vi "Set Description.vi"(8 "error in":errorcluster, 11 "ILabVIEWFile in":refnum<class "Type Definition.lvclass">) -> (0 "error out":errorcluster, 3 "ILabVIEWFile out":refnum<class "Type Definition.lvclass">)   [LabVIEW 2026, in "Type Definition.lvclass"]
doc: "Set description of labview file (vi or type definition)."
uses:
  Type Definition.lvclass
  Type Definition.lvclass/Type Definition.ctl
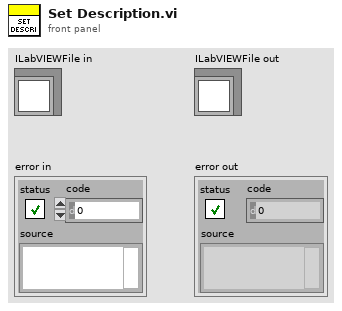
[diagram p1: front panel]
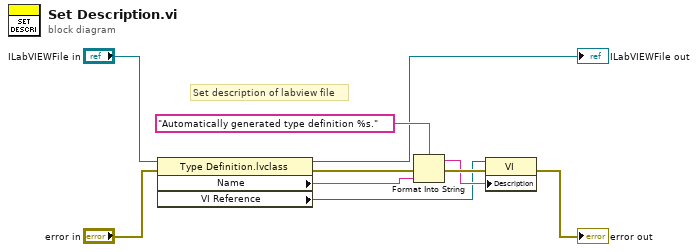
[diagram p0: block diagram]
diagram:
  # "Set description of labview file"
  n1 = property class="Type Definition.lvclass"(reference="ILabVIEWFile in", error in="error in") -> (reference out=→"ILabVIEWFile out":refnum<class "Type Definition.lvclass">, error out=w7:errorcluster, "Name"=w3:string, "VI Reference"=w1:refnum<vi>)
  n2 = Format Into String(format string="Automatically generated type definition %s.", error in=w7, w3) -> (resulting string=w5:string, error out=w9:errorcluster)  [unwired: 1 in]
  n3 = property on="Property Node" class="VI"(reference=w1, error in=w9, "Description"=w5) -> (error out=→"error out":errorcluster)  [unwired: 1 out]
